vi "Traverse Get Positions.vi"(8 "error in":errorcluster, 10 "VISA resource name":refnum<visa-resource-name>, 11 "Water Tunnel Results in":refnum<class "Water Tunnel Results.lvclass">) -> (0 "error out":errorcluster, 1 "Trav Probe":cluster{"Pz":dbl}, 2 "Trav Wing":cluster{"Wx":dbl, "Wz":dbl, "Wa":dbl}, 3 "Water Tunnel Results out":refnum<class "Water Tunnel Results.lvclass">)   [LabVIEW 2019, in "Results.lvlib" / "Water Tunnel Results.lvclass"]
uses:
  Water Tunnel Results.lvclass
  Water Tunnel Results.lvclass/Water Tunnel Results.ctl
  e4db5d3b-805d-4592-a1bd-8ead1afbec68.vi
panel:
  out "Traverse Message":string
  out "Traverse Raw String":string
  out "Count X":u32
  out "Count Y":u32
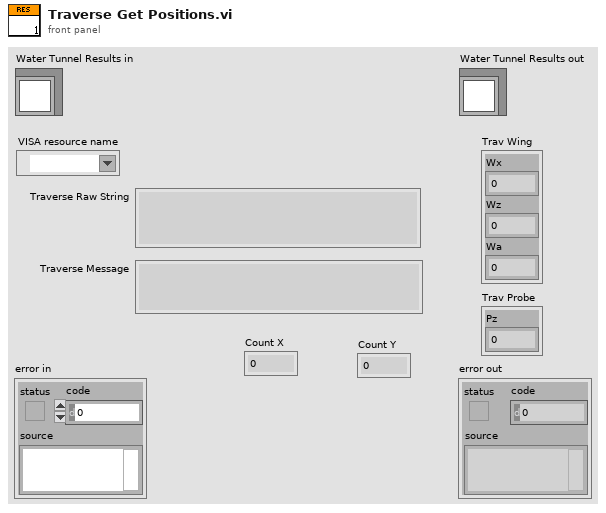
[diagram p1: front panel]
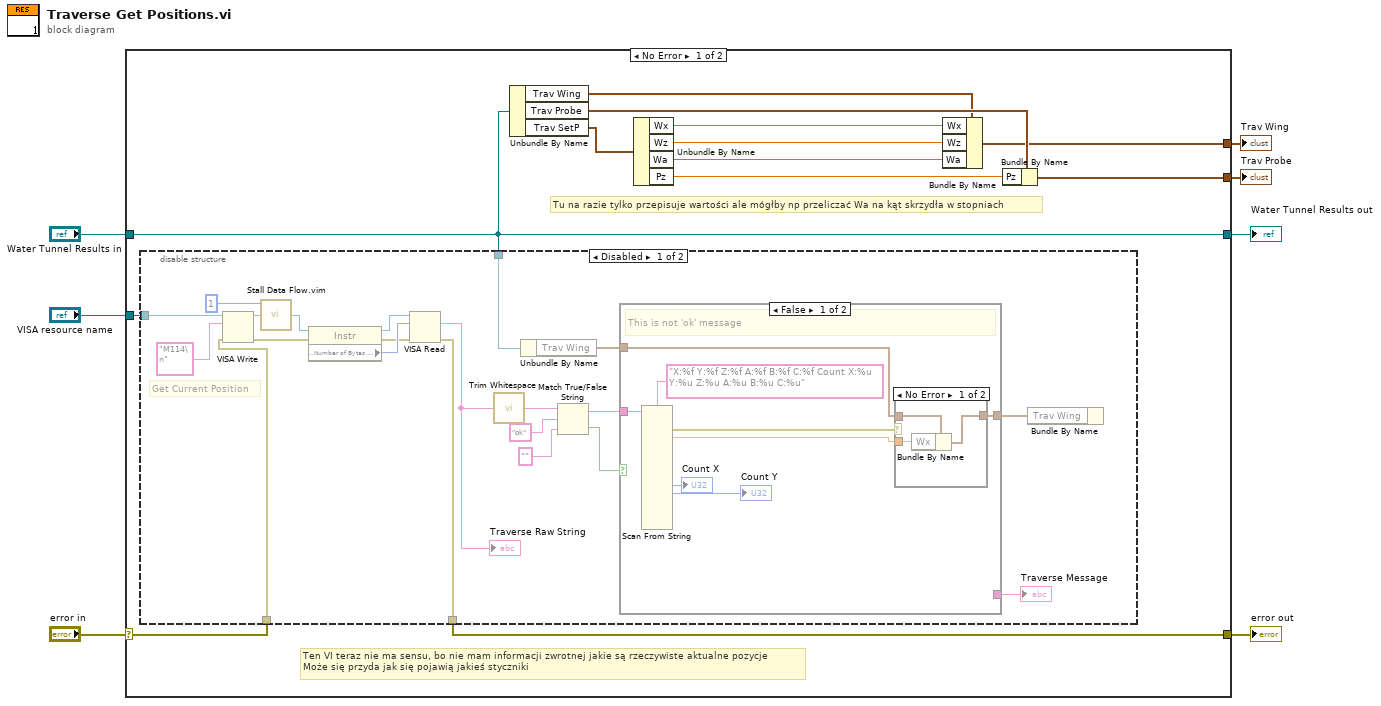
[diagram p0: block diagram]
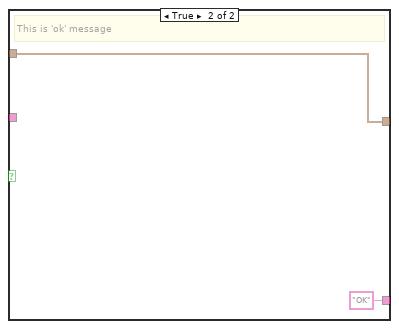
[diagram p3: hidden frame]
diagram:
  n1 = case shown="No Error" "error in" {
    selector: "error in" -> [w8 w58]
    tunnel: [w19 w58] -> w6
    tunnel: [w18 w57] -> w4
    tunnel: "Water Tunnel Results in" -> [w18 w57]
    tunnel: "VISA resource name" -> [w20 _]
    tunnel: [w10 _] -> w1
    tunnel: [w9 _] -> w2
    frame No Error {
      # "Tu na razie tylko przepisuje wartości ale mógłby np przeliczać Wa na kąt skrzydła w stopniach"
      # "Ten VI teraz nie ma sensu, bo nie mam informacji zwrotnej jakie są rzeczywiste aktualne pozycje\nMoże się przyda jak się pojawią jakieś styczniki"
      n2 = disable-structure shown="Disabled" {
        disable-tunnel: w20 -> [w37 _]
        disable-tunnel: [w35 w56] -> w19
        disable-tunnel: w18 -> [w22 _]
        disable-tunnel: w8 -> [w21 w56]
        frame Disabled {
          # "Get Current Position"
          n3 = VISA Write(VISA resource name=w37, write buffer="M114\n", error in (no error)=w21) -> (VISA resource name out=w34:refnum<visa-resource-name>, error out=w38:errorcluster)  [unwired: 1 out]
          n4 = call "Stall Data Flow.vim"("value in"=w34, "milliseconds to wait"=u32 1) -> ("value out"=w33:refnum<visa-resource-name>)  [unwired: 1 out]
          n5 = property class="Instr"(reference=w33, error in=w38) -> (reference out=w41:refnum<visa-resource-name>, error out=w39:errorcluster, "Serial Settings:Number of Bytes at Serial Port"=w40:u32)
          n6 = VISA Read(VISA resource name=w41, byte count=w40, error in (no error)=w39) -> (read buffer=w24:string, error out=w35:errorcluster)  [unwired: 2 out]
          "Traverse Raw String" <- w24
          n7 = call <vilib>:"Trim Whitespace.vi"("string"=w24) -> ("trimmed string"=w31:string)  [unwired: 1 in]
          n8 = Unbundle By Name(w22) -> ("Trav Wing"=w26:cluster{"Wx":dbl, "Wz":dbl, "Wa":dbl})
          n9 = Match True/False String(2:"" ("false string"), 3:"ok" ("true string"), 4:w31) -> (0:w29:bool, 1:w28:string)
          n10 = case shown="False" w29 {
            tunnel: w28 -> [w46 _]
            tunnel: w26 -> [w45 w55]
            tunnel: [w42 w55] -> w25
            tunnel: [_ "OK" ("trimmed string")] -> w23
            frame False {
              # "This is not 'ok' message"
              n11 = Scan From String(format string="X:%f Y:%f Z:%f A:%f B:%f C:%f Count X:%u Y:%u Z:%u A:%u B:%u C:%u", input string=w46) -> (error out=w43:errorcluster, output 1=w44:dbl, output 7=→"Count X":u32, output 8=→"Count Y":u32)  [unwired: 23 in, 2 out]
              n12 = case shown="No Error" w43 {
                tunnel: w45 -> [w52 w53]
                tunnel: w44 -> [w51 _]
                tunnel: [w50 w53] -> w42
                frame No Error {
                  n13 = Bundle By Name(cluster=w52, "Wx"=w51) -> (w50:cluster{"Wx":dbl, "Wz":dbl, "Wa":dbl})
                }
                frame Error {
                }
              }
            }
            frame True {
              # "This is 'ok' message"
            }
          }
          "Traverse Message" <- w23
          n14 = Bundle By Name("Trav Wing"=w25) -> ()  [unwired: 1 in, 1 out]
        }
        frame Enabled {
        }
      }
      n15 = Unbundle By Name(w18) -> ("Trav Wing"=w15:cluster{"Wx":dbl, "Wz":dbl, "Wa":dbl}, "Trav Probe"=w16:cluster{"Pz":dbl}, "Trav SetP"=w17:cluster{"Wx":dbl, "Wz":dbl, "Wa":dbl, "Pz":dbl})
      n16 = Unbundle By Name(w17) -> ("Wx"=w14:dbl, "Wz"=w13:dbl, "Wa"=w12:dbl, "Pz"=w11:dbl)
      n17 = Bundle By Name(cluster=w15, "Wx"=w14, "Wz"=w13, "Wa"=w12) -> (w10:cluster{"Wx":dbl, "Wz":dbl, "Wa":dbl})
      n18 = Bundle By Name(cluster=w16, "Pz"=w11) -> (w9:cluster{"Pz":dbl})
    }
    frame Error {
    }
  }
  "error out" <- w6
  "Water Tunnel Results out" <- w4
  "Trav Probe" <- w2
  "Trav Wing" <- w1
